vi "Hatch Control.vi"(10 "Driver Right Bumper":bool, 11 "Driver Left Bumper":bool) -> (3 "Hatch Intake Floor":dbl)   [LabVIEW 2018]
uses:
  Infrastructure/Constants.vi
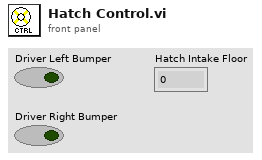
[diagram p1: front panel]
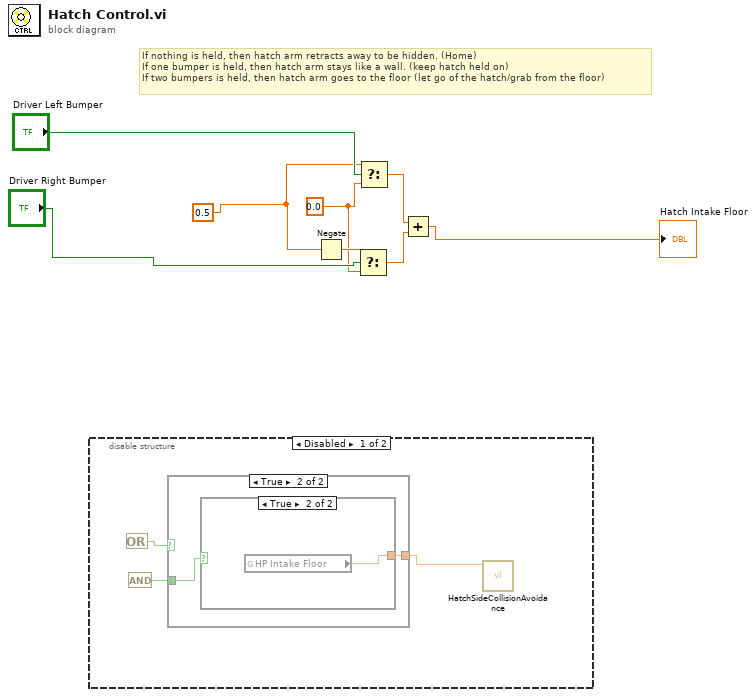
[diagram p0: block diagram]
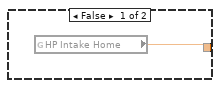
[diagram p2: hidden frame]
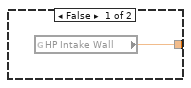
[diagram p3: hidden frame]
diagram:
  w2 = 0.5
  w5 = 0.0
  # "If nothing is held, then hatch arm retracts away to be hidden. (Home)\nIf one bumper is held, then hatch arm stays like a wall. (keep hatch held on)\nIf two bumpers is held, then hatch arm goes to the floor (let go of the hatch/grab from the floor)"
  n1 = disable-structure shown="Disabled" {
    frame Disabled {
      n2 = Or() -> (x .or. y?=w10:bool)  [unwired: 2 in]
      n3 = And() -> (x .and. y?=w9:bool)  [unwired: 2 in]
      n4 = case shown="True" w10 {
        tunnel: w9 -> [_ w14]
        tunnel: [w12 w13] -> w11
        frame False {
          n5 = global read "Constants.vi" "HP Intake Home"() -> (w12:dbl)
        }
        frame True {
          n6 = case shown="True" w14 {
            tunnel: [w15 w16] -> w13
            frame False {
              n7 = global read "Constants.vi" "HP Intake Wall"() -> (w15:dbl)
            }
            frame True {
              n8 = global read "Constants.vi" "HP Intake Floor"() -> (w16:dbl)
            }
          }
        }
      }
      n9 = call "HatchSideCollisionAvoidance.vi"("Intended Hatch Setpoint"=w11) -> ()  [unwired: 10 in, 1 out]
    }
    frame Enabled {
    }
  }
  n10 = Negate(x=w2) -> (-x=w6:dbl)
  n11 = Select(t=w6, s="Driver Right Bumper", f=w5) -> (s? t:f=w4:dbl)
  n12 = Select(t=w2, s="Driver Left Bumper", f=w5) -> (s? t:f=w3:dbl)
  n13 = Add(x=w3, y=w4) -> (x+y=→"Hatch Intake Floor":dbl)
